vi "Draw Price Chart.vi"(10 "title":string, 11 "prices":dbl[](array[numeric])) -> (3 "chart":picture)   [LabVIEW 2020, in "Full Featured MCP Server.lvlib"]
doc: "Draws a price curve as a picture with Plot Waveform.vi: the x axis counts seconds and ends at 0 = now, the y axis is scaled to the lowest and highest price shown. The title is written above the plot."
uses:
  Full Featured MCP Server.lvlib
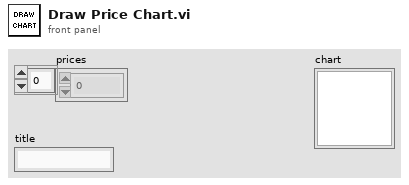
[diagram p1: front panel]
types:
  T1 = cluster{"plot color":u32, "waveform plot type":enum16{"points", "squares", "circles", "connected points", "connected squares", "connected circles", "fill to baseline", "comb plot", "bar plot"}, "baseline":dbl}
  T2 = cluster{"line color":u32, "text color":u32, "tick length(3)":i16, "crossing axes":bool, "visible grid?":bool}
  T3 = cluster{"left":i16, "top":i16, "right":i16, "bottom":i16}
  T4 = cluster{"Xo(0)":dbl, "delta X(1)":dbl, "Y data":dbl[]}
  T5 = cluster{"x minimum":dbl, "x maximum":dbl, "x log?":bool, "x precision":u8, "x format":enum8{"Decimal", "Scientific", "Engineering", "Binary", "Octal", "Hex"}, "y minimum":dbl, "y maximum":dbl, "y log?":bool, "y precision":u8, "y format":enum8{"Decimal", "Scientific", "Engineering", "Binary", "Octal", "Hex"}}
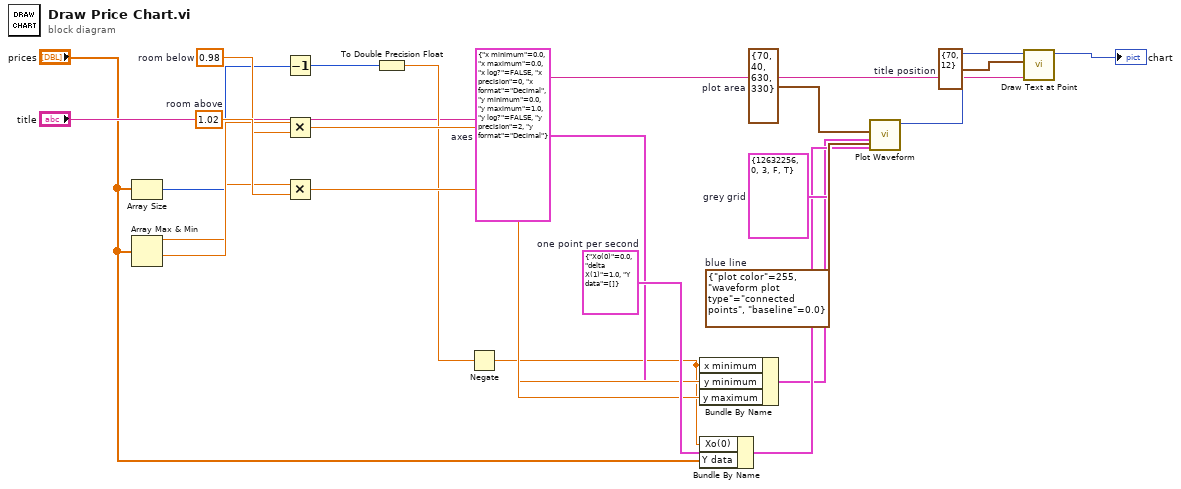
[diagram p0: block diagram]
diagram:
  w21 = cluster{"x":i16, "y":i16} {"x"=70, "y"=12}  # title position
  w19 = T1 {"plot color"=255, "waveform plot type"=enum."connected points", "baseline"=0.0}  # blue line
  w18 = T2 {"line color"=12632256, "text color"=0, "tick length(3)"=3, "crossing axes"=FALSE, "visible grid?"=TRUE}  # grey grid
  w17 = T3 {"left"=70, "top"=40, "right"=630, "bottom"=330}  # plot area
  w15 = T4 {"Xo(0)"=0.0, "delta X(1)"=1.0, "Y data"=[]}  # one point per second
  w12 = 1.02  # room above
  w10 = 0.98  # room below
  w9 = T5 {"x minimum"=0.0, "x maximum"=0.0, "x log?"=FALSE, "x precision"=0, "x format"=enum."Decimal", "y minimum"=0.0, "y maximum"=1.0, "y log?"=FALSE, "y precision"=2, "y format"=enum."Decimal"}  # axes
  n1 = Array Size(array="prices") -> (size(s)=w3:i32)
  n2 = Array Max & Min(array="prices") -> (max value=w7:dbl, min value=w8:dbl)  [unwired: 2 out]
  n3 = Decrement(x=w3) -> (x-1=w4:i32)
  n4 = Multiply(x=w8, y=w10) -> (x*y=w11:dbl)
  n5 = Multiply(x=w7, y=w12) -> (x*y=w13:dbl)
  n6 = To Double Precision Float(number=w4) -> (double precision float=w5:dbl)
  n7 = Negate(x=w5) -> (-x=w6:dbl)
  n8 = Bundle By Name(cluster=w9, "x minimum"=w6, "y minimum"=w11, "y maximum"=w13) -> (w14:T5)
  n9 = Bundle By Name(cluster=w15, "Xo(0)"=w6, "Y data"="prices") -> (w16:T4)
  n10 = call <vilib>:"Plot Waveform.vi"("waveform plot cosmetics"=w19, "cartesian grid cosmetics"=w18, "waveform data"=w16, "cartesian axis attributes"=w14, "bounding rect"=w17) -> ("new picture"=w20:picture)  [unwired: 6 in]
  n11 = call <vilib>:"Draw Text at Point.vi"("text"="title", "origin"=w21, "picture"=w20) -> ("new picture"=→"chart":picture)  [unwired: 7 in, 1 out]
